vi "Brown--constant.vi"() -> (1 "Brown":u32(colorbox))   [LabVIEW 2018, in "Band Colors.lvlib"]
doc: "Provides the RGB color value for brown.\n\nThe VI converts the RGB components (120, 72, 0) into a LabVIEW color value and returns it through <b>Brown</b>."
uses:
  Band Colors.lvlib
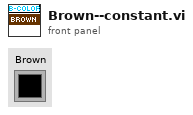
[diagram p1: front panel]
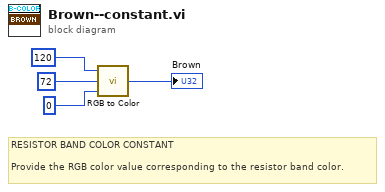
[diagram p0: block diagram]
diagram:
  # "RESISTOR BAND COLOR CONSTANT\n\nProvide the RGB color value corresponding to the resistor band color."
  n1 = call <vilib>:"RGB to Color.vi"("B"=u8 0, "G"=u8 72, "R"=u8 120) -> ("Color"=→"Brown":u32)
